vi "ZM-PC-TP-create.vi"(8 "error in (no error)":errorcluster, 10 "data":T1) -> (0 "error out":errorcluster, 3 "package":refnum<class "ZM-PC-TP-test_package.lvclass">)   [LabVIEW 2020, in "ZM-PC-packages.lvlib" / "ZM-PC-TP-test_package.lvclass"]
doc: "Creates a test package: a default ZM-PC-TP-test_package object, initialised by ZM-PC-init (dynamic, so the child's override sets timestamp and type), then the data cluster written through Write data. Static, public: the creator's entry point."
uses:
  ZM-PC-TP-test_package.lvclass
  ZM-PC-TP-test_package.lvclass/ZM-PC-TP-test_package.ctl
  ZM-PC-TP-DATA.ctl
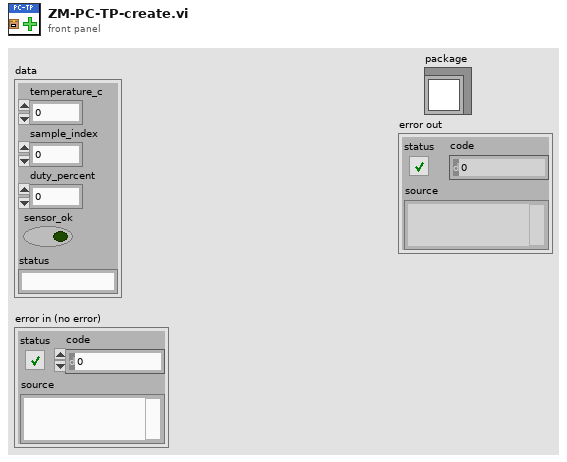
[diagram p1: front panel]
types:
  T1 = typedef "ZM-PC-packages.lvlib/ZM-PC-TP-test_package.lvclass/ZM-PC-TP-DATA.ctl" = cluster{"temperature_c":dbl, "sample_index":i32, "duty_percent":u8, "sensor_ok":bool, "status":string}
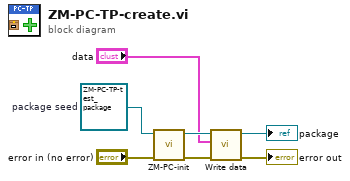
[diagram p0: block diagram]
diagram:
  w7 = refnum<class "ZM-PC-TP-test_package.lvclass"> refnum  # package seed
  n1 = call-dynamic "ZM-PC-init.vi"("error in (no error)"="error in (no error)", "ZM-PC-TP-test_package in"=w7) -> ("error out"=w5:errorcluster, "ZM-PC-TP-test_package out"=w4:refnum<class "ZM-PC-TP-test_package.lvclass">)  [unwired: 8 in]
  n2 = call "Write data.vi"("error in (no error)"=w5, "ZM-PC-TP-DATA"="data", "ZM-PC-TP-test_package in"=w4) -> ("error out"=→"error out":errorcluster, "ZM-PC-TP-test_package out"=→"package":refnum<class "ZM-PC-TP-test_package.lvclass">)  [unwired: 7 in]
